vi "CalcExpress Light.vi"(5 "directives":T1={"enaNamedConst"=TRUE}, 7 "VC Handle":T5=-1, 8 "error in":bool, 9 "params":T3={"autoVar"=TRUE, "enCpx"=TRUE}, 10 "repeat (1)":i32=1, 11 "expression":string) -> (0 "error out":bool, 1 "value type":T4=enum."DBL Number", 3 "numeric value":dbl, 4 "error description":string)   [LabVIEW 2021]
doc: "The VI evaluates CalcExpress expressions and sequential scripts. To process non-sequential scripts involving loops and branches, use CSE VIs.\n\n<B>VC Handle</B> should contain handle of variable context. Variables of the corresponding context can be used in an expression.\n\n<B>repeat</B> control determines number of times an expression needs to be evaluated. By default, it is equal to one (1).\n\n<B>params</B> cluster specifies optional parameters influencing on evaluation.\n params.autoVar - If it's TRUE (by default) and there is a reference to unexistent variable on the left side of an assignment operator, CalcExpress implicitly creates the variable. If it's FALSE, all variables referenced in a script must be explicitly created either before or during evaluation.\n params.enCpx parameter enables or disables performing operators on operands of non-Numeric types (TRUE by default).\n\nFor more information, see help for this VI.\n\n::: CalcExpress Toolkit :::\nCopyright (c) 2000-2026 Konstantin Shifershteyn. All rights reserved."
uses:
  cetypes.llb/VarMan Variable Context Handle.ctl
  cetypes.llb/CalcExpress Data Type.ctl
  cetypes.llb/CalcExpress Execution Options.ctl
  cetypes.llb/CalcExpress Instance RefNum.ctl
  cetypes.llb/CalcExpress Parsing Directives.ctl
  cersrc/celveng32.dll
panel:
  in  "CE InstanceRef":T2
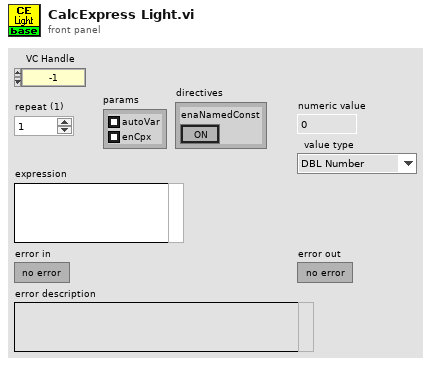
[diagram p1: front panel]
types:
  T1 = typedef "CalcExpress Parsing Directives.ctl" = cluster{"enaNamedConst":bool}
  T2 = typedef "CalcExpress Instance RefNum.ctl" = refnum<k1>
  T3 = typedef "CalcExpress Execution Options.ctl" = cluster{"autoVar":bool, "enCpx":bool}
  T4 = typedef "CalcExpress Data Type.ctl" = enum32{"String", "DBL Number", "identifier", "1D Array of DBL", "2D Array of DBL", "CDB Number", "1D Array of CDB", "2D Array of CDB", "1D Array of String", "2D Array of String", "Unknown data type"}
  T5 = typedef "VarMan Variable Context Handle.ctl" = i32
  T6 = enum32{"String", "DBL Number", "identifier", "1D Array of DBL", "2D Array of DBL", "CDB Number", "1D Array of CDB", "2D Array of CDB", "1D Array of String", "2D Array of String", "Unknown data type"}
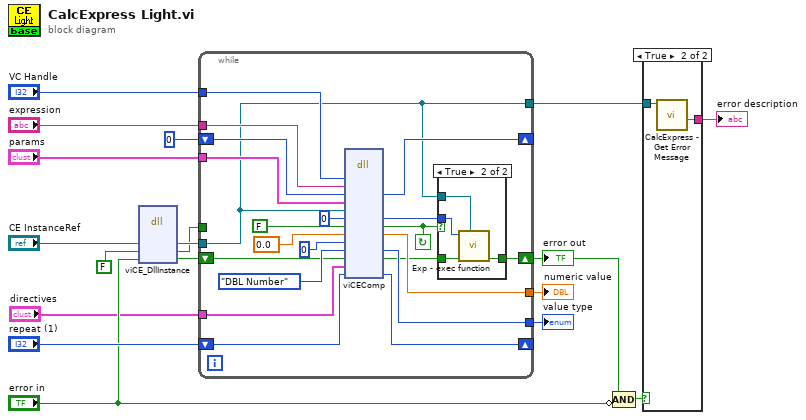
[diagram p0: block diagram]
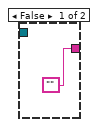
[diagram p3: hidden frame]
diagram:
  n1 = dll-call lib="C:/LV Projects/CalcExpress 40 LV2021/vi.lib/addons/CalcExpress/cersrc/celveng*.dll" fn="viCE_DllInstance"("iRef"="CE InstanceRef", "newInst"=FALSE, "err_f"="error in") -> ("iRef"=w10:T2, "newInst"=w2:bool, "err_f"=w11:bool)  [unwired: 6 in, 2 out]
  n2 = while {
    tunnel: [w24] -> w5
    shift-left: "repeat (1)" -> [w21]
    shift-right: [w20] -> _
    tunnel: [w25] -> w14
    tunnel: [w28] -> w15
    tunnel: w10 -> [w24]
    tunnel: "expression" -> [w37]
    tunnel: "VC Handle" -> [w38]
    tunnel: "params" -> [w34]
    shift-left: 0 -> [w36]
    shift-right: [w35] -> _
    shift-left: w11 -> [w23]
    shift-right: [w39] -> w7
    tunnel: w2 -> [_]
    tunnel: "directives" -> [w19]
    stop <- w30 continue-if-true
    n3 = dll-call lib="C:/LV Projects/CalcExpress 40 LV2021/vi.lib/addons/CalcExpress/cersrc/celveng*.dll" fn="viCEComp"("vch"=w38, "script"=w37, "idx"=w36, "cPar"=w34, "iRef"=w24, "opdNum"=0, "NE"=FALSE, "num"=0.0, "str"=u64 0, "type"=T6."DBL Number" ("data type"), "erf"=w23, "dirs"=w19, "rept"=w21) -> ("idx"=w35:i32, "opdNum"=w32:i32, "NE"=w30:bool, "num"=w28:dbl, "type"=w25:T6, "erf"=w22:bool, "rept"=w20:i32)  [unwired: 10 in, 2 out]
    n4 = case shown="True" w30 {
      tunnel: [w40 w44] -> w39
      tunnel: w22 -> [w40 w43]
      tunnel: w32 -> [_ w42]
      tunnel: w24 -> [_ w41]
      frame False {
      }
      frame True {
        n5 = call "Exp - exec function.vi"("CE InstanceRef"=w41, "error in"=w43, "ParNum"=w42) -> ("error out"=w44:bool)  [unwired: 6 in]
      }
    }
  }
  "error out" <- w7
  "numeric value" <- w15
  "value type" <- w14
  n6 = Compound Arithmetic op=AND(w7, invert "error in") -> (w6:bool)
  n7 = case shown="True" w6 {
    tunnel: w5 -> [_ w47]
    tunnel: ["" w46] -> w3
    frame False {
    }
    frame True {
      n8 = call "CalcExpress - Get Error Message.vi"("CE InstanceRef"=w47) -> ("error description"=w46:string)  [unwired: 5 in, 3 out]
    }
  }
  "error description" <- w3
